vi "RT Functions v03a CMA w TS_Meas.vi"(7 "Function":T5(ring)=enum."CS_Measure", 8 "error in (no error)":errorcluster, 9 "DAQ Trigger":T4={"Trig Source"=0, "Digital Trigger"=FALSE, "Trig Edge"=10171, "Pulse Line"=0, "Pulse On Time"=0} {"Pulse Line" items=["/Line0", "/Line1", "/Line2", "/Line3", "/Line4", "/Line5", "/Line6", "/Line7", "/Line8", "/Line9", "/Line10", "/Line11", "/Line12", "/Line13", "/Line14", "/Line15"]; "Trig Edge" items=["Rising"=10280, "Falling"=10171]; "Trig Source" items=["PFI0", "PFI1", "PFI2", "PFI3", "PFI4", "PFI5", "PFI6", "PFI7", "PFI8", "PFI9", "PFI10", "PFI11", "PFI12", "PFI13", "PFI14", "PFI15"]}, 10 "DAQ Timing":T3={"Number of Samples"=40000, "Samples Per Second"=970000.0, "Sample Mode"=10178, "Timeout (s)"=10.0} {"Sample Mode" items=["Continuous"=10123, "Finite Sample"=10178, "Hardware Timed Single Point"=12522]}, 11 "DAQ Channel":T2={"Channel"=1, "input terminal configuration"=10106, "Input Range Range"=10.0, "Device"="DAQ1"} {"input terminal configuration" items=["default"=-1, "RSE"=10083, "NRSE"=10078, "Differential"=10106, "Pseudodifferential"=12529]; "Input Range Range" items=["+/-10V"=10.0, "+/-5V"=5.0, "+/-2V"=2.0, "+/-1V"=1.0, "+/-0.5V"=0.5, "+/-0.2V"=0.2, "+/-0.1V"=0.1]; "Channel" items=["0"=0, "1"=1, "2"=2, "3"=3, "4"=4, "5"=5, "6"=6, "7"=7, "8"=8, "9"=9, "10"=10, "11"=11, "12"=12, "13"=13, "14"=14, "15"=15, "16"=16, "17"=18, "19"=20, "21"=22, "23"=24, "25"=26, "27"=28, "29"=30, "31"=32]}) -> (0 "error out":errorcluster, 2 "Wfm":waveform(dbl)={"t0"=timestamp(3404415606.9661703 s since 1904-01-01), "dt"=1.0299999999999546e-06, "Y"=array[1600 elements], "attributes"=variant("NI_ChannelName"=variant(string "Voltage"), "NI_UnitDescription"=variant(string "Volts"))}, 3 "Mean":dbl format="%0.2f", 6 "DAQ Pusle":T1)   [LabVIEW 2013]
uses:
  <vilib>/Analysis/baseanly.llb/Mean (DBL).vi
  <vilib>/Waveform/WDTOps.llb/WDT Get Waveform Subset DBL.vi
  <vilib>/Analysis/NI_AALBase.lvlib
panel:
  out "V1_Wfm 2":waveform(dbl)
  out "V2_Wfm 2":waveform(dbl)
  out "V3_Wfm":waveform(dbl)
  out "V2_Wfm":waveform(dbl)
  out "V1_Wfm":waveform(dbl)
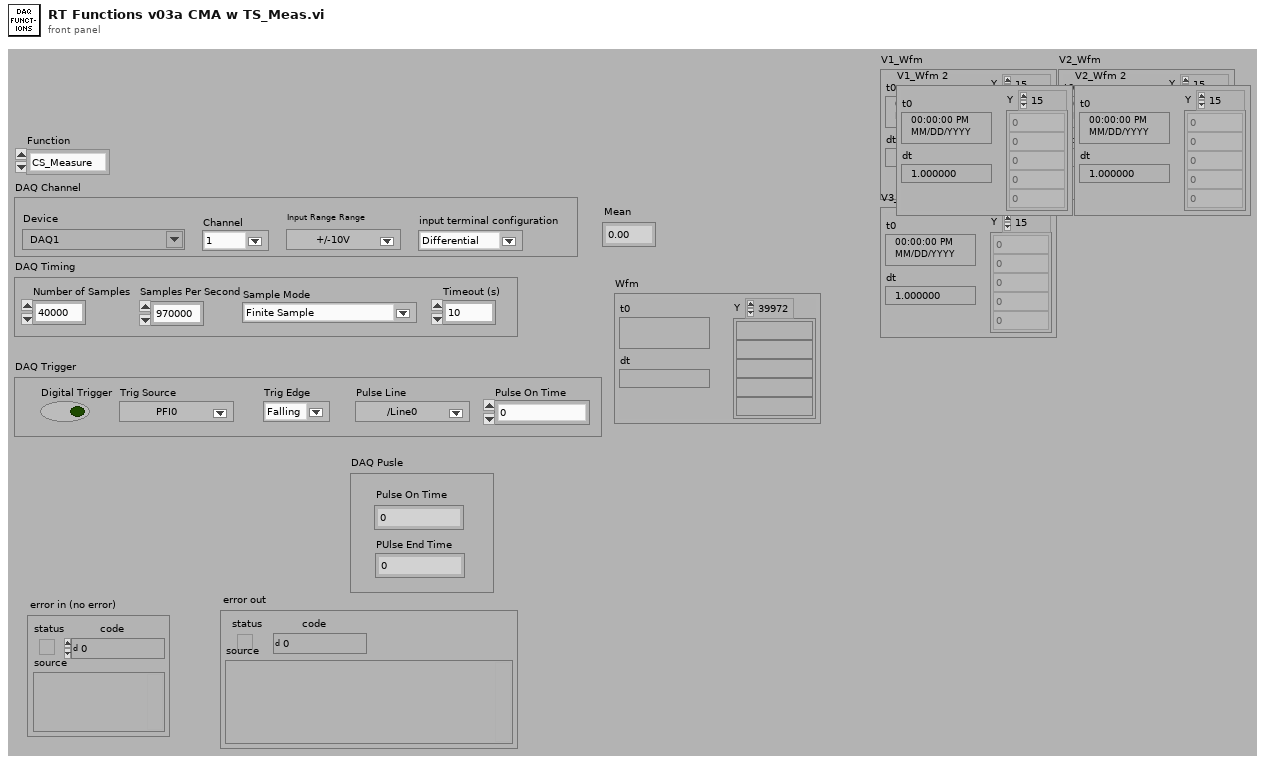
[diagram p1: front panel]
types:
  T1 = cluster{"Pulse On Time":u32, "PUlse End Time":u32}
  T2 = cluster{"Channel":u16, "input terminal configuration":i32, "Input Range Range":dbl, "Device":string}
  T3 = cluster{"Number of Samples":u32, "Samples Per Second":dbl, "Sample Mode":i32, "Timeout (s)":dbl}
  T4 = cluster{"Trig Source":u16, "Digital Trigger":bool, "Trig Edge":i32, "Pulse Line":u16, "Pulse On Time":u32}
  T5 = enum32{"V1 Measure", "V2 Measure", "V3 Measure", "CS_Measure", "TS_Measure", "Pulse On", "Pulse Off"}
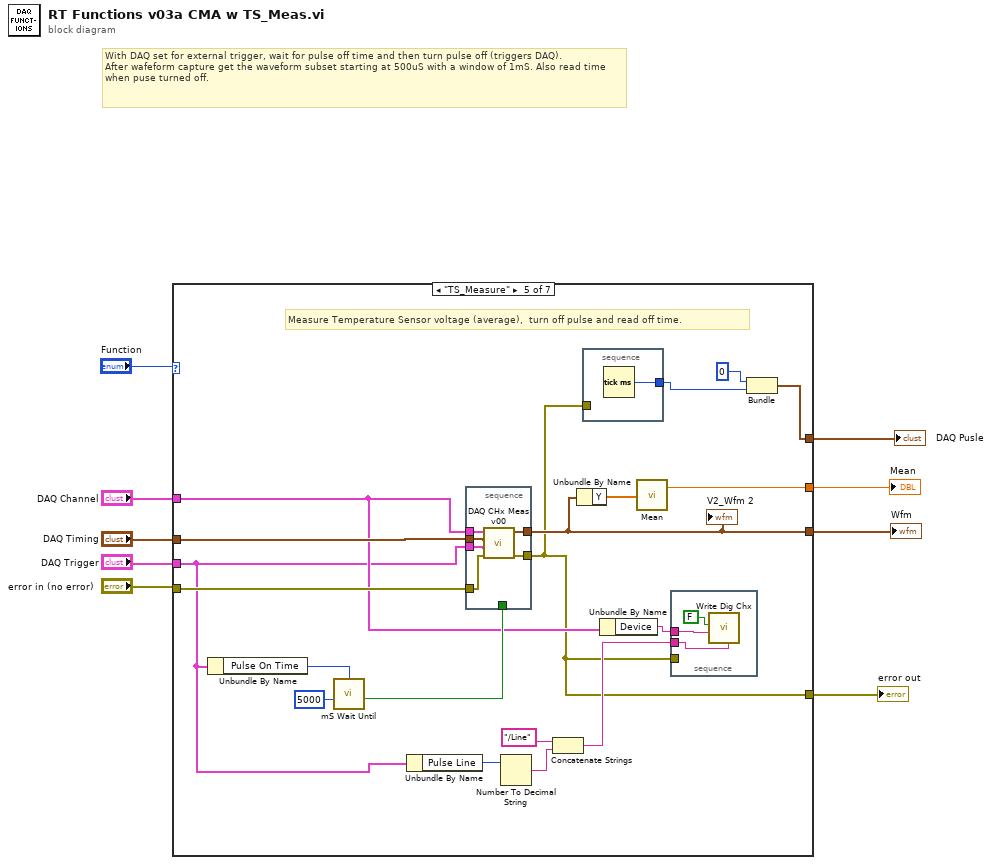
[diagram p0: block diagram]
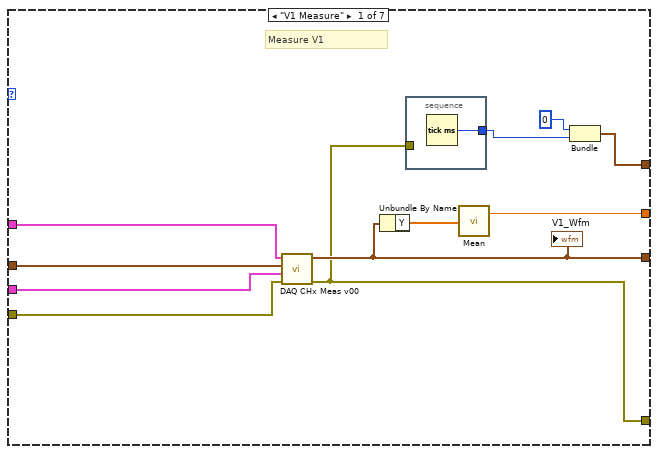
[diagram p2: hidden frame]
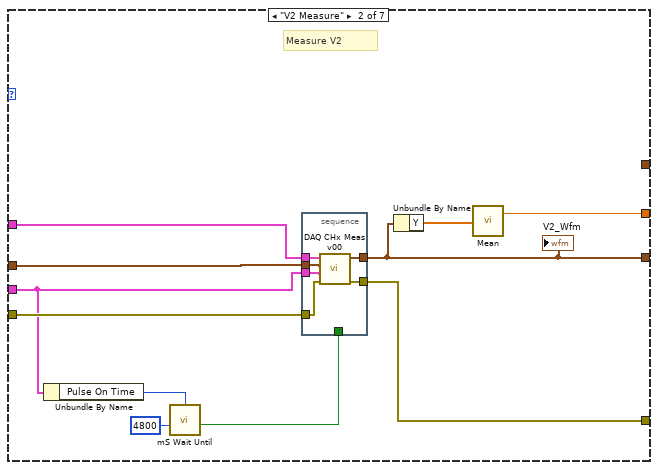
[diagram p3: hidden frame]
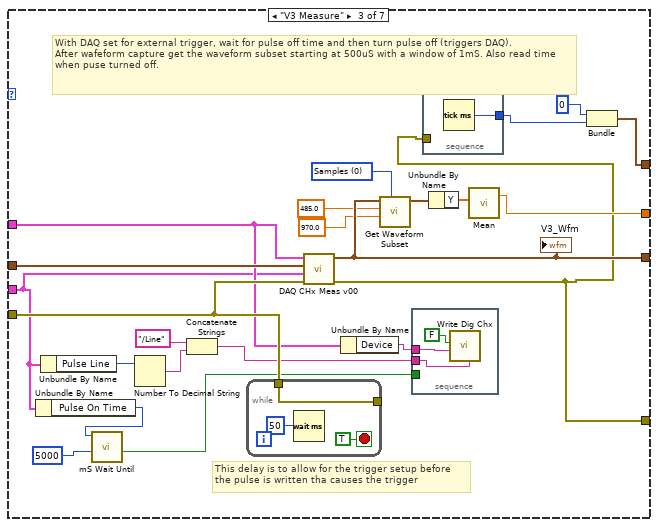
[diagram p4: hidden frame]
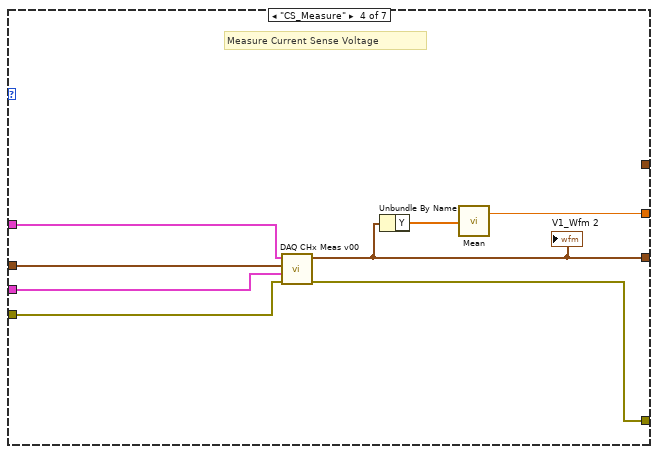
[diagram p5: hidden frame]
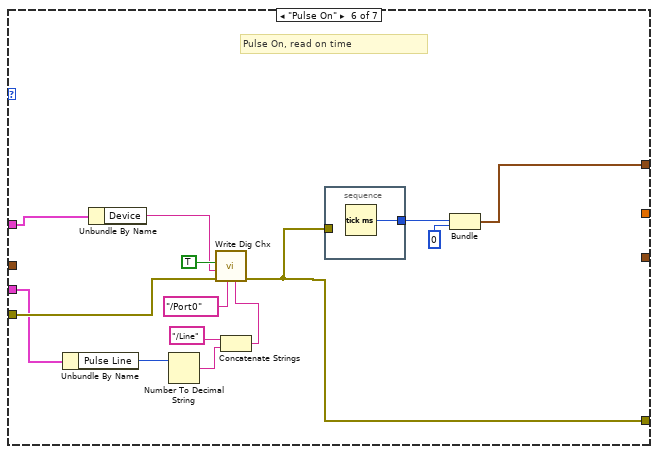
[diagram p6: hidden frame]
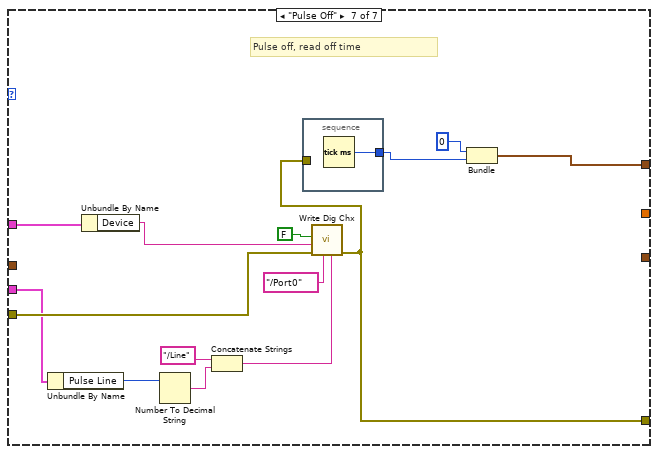
[diagram p7: hidden frame]
diagram:
  # "With DAQ set for external trigger, wait for pulse off time and then turn pulse off (triggers DAQ).\nAfter wafeform capture get the waveform subset starting at 500uS with a window of 1mS. Also read time when puse turned off."
  n1 = case shown="\"TS_Measure\"" "Function" {
    tunnel: "error in (no error)" -> [w20 w31 w58 w76 w95 w118 w133]
    tunnel: [w10 w32 w39 w75 w77 w114 w129] -> w8
    tunnel: "DAQ Channel" -> [w14 w26 w57 w69 w86 w117 w132]
    tunnel: "DAQ Timing" -> [w19 w30 w61 w74 w94 _ _]
    tunnel: "DAQ Trigger" -> [w18 w22 w43 w73 w82 w109 w124]
    tunnel: [w17 w28 w55 w72 w92 _ _] -> w3
    tunnel: [w15 w27 w59 w70 w91 _ _] -> w2
    tunnel: [w11 _ w40 _ w78 w106 w123] -> w1
    frame "V1 Measure" {
      # "Measure V1"
      n2 = call "DAQ CHx Meas v00.vi"("error in"=w20, "DAQ Trigger"=w18, "DAQ Timing"=w19, "DAQ Channel"=w14) -> ("error out"=w10:errorcluster, "Waveform"=w17:waveform(dbl))  [unwired: 6 in]
      "V1_Wfm" <- w17
      n3 = Unbundle By Name(w17) -> ("Y"=w16:dbl[])
      n4 = stacked-sequence {
        tunnel: [w21] -> w13
        tunnel: w10 -> [_]
        frame #0 {
          n5 = Tick Count (ms)() -> (millisecond timer value=w21:u32)
        }
      }
      n6 = call-poly <vilib>:"Mean.vi"("X"=w16) -> ("mean"=w15:dbl)  [unwired: 1 out]
      n7 = Bundle(u32 0, "millisecond timer value"=w13) -> (w11:cluster{u32, "millisecond timer value":u32})  [unwired: 1 in]
    }
    frame "V2 Measure" {
      # "Measure V2"
      n8 = Unbundle By Name(w22) -> ("Pulse On Time"=w23:u32)
      n9 = call "mS Wait Until.vi"("mS Delta"=u16 4800, "mS Start Time"=w23) -> ("Done"=w24:bool)  [unwired: 8 in, 1 out]
      n10 = stacked-sequence {
        tunnel: [w38] -> w32
        tunnel: w31 -> [w37]
        tunnel: w30 -> [w36]
        tunnel: w22 -> [w35]
        tunnel: [w34] -> w28
        tunnel: w26 -> [w33]
        tunnel: w24 -> [_]
        frame #0 {
          n11 = call "DAQ CHx Meas v00.vi"("error in"=w37, "DAQ Trigger"=w35, "DAQ Timing"=w36, "DAQ Channel"=w33) -> ("error out"=w38:errorcluster, "Waveform"=w34:waveform(dbl))  [unwired: 6 in]
        }
      }
      "V2_Wfm" <- w28
      n12 = Unbundle By Name(w28) -> ("Y"=w29:dbl[])
      n13 = call-poly <vilib>:"Mean.vi"("X"=w29) -> ("mean"=w27:dbl)  [unwired: 1 out]
    }
    frame "V3 Measure" {
      w54 = u16 0 items=["Samples", "Relative Time"] ("start/duration format")
      # "With DAQ set for external trigger, wait for pulse off time and then turn pulse off (triggers DAQ).\nAfter wafeform capture get the waveform subset starting at 500uS with a window of 1mS. Also read time when puse turned off."
      # "This delay is to allow for the trigger setup before\nthe pulse is written tha causes the trigger"
      n14 = Unbundle By Name(w43) -> ("Pulse On Time"=w48:u32)
      n15 = Unbundle By Name(w43) -> ("Pulse Line"=w47:u16)
      n16 = call "mS Wait Until.vi"("mS Delta"=u16 5000, "mS Start Time"=w48) -> ("Done"=w49:bool)  [unwired: 8 in, 1 out]
      n17 = Number To Decimal String(number=w47) -> (decimal integer string=w46:string)  [unwired: 1 in]
      n18 = Concatenate Strings("/Line", w46) -> (w44:string)
      n19 = while {
        tunnel: w58 -> [w66]
        tunnel: [w66] -> _
        stop <- TRUE stop-if-true
        n20 = Wait (ms)(milliseconds to wait=u32 50) -> ()  [unwired: 1 out]
      }
      n21 = call "DAQ CHx Meas v00.vi"("error in"=w58, "DAQ Trigger"=w43, "DAQ Timing"=w61, "DAQ Channel"=w57) -> ("error out"=w39:errorcluster, "Waveform"=w55:waveform(dbl))  [unwired: 6 in]
      "V3_Wfm" <- w55
      n22 = Unbundle By Name(w57) -> ("Device"=w56:string)
      n23 = call-poly <vilib>:"Get Waveform Subset.vi"("start/duration format"=w54, "duration"=970.0, "start samples/time"=485.0, "waveform in"=w55) -> ("waveform out"=w51:waveform(dbl))  [unwired: 2 in, 3 out]
      n24 = stacked-sequence {
        tunnel: w56 -> [w64]
        tunnel: w44 -> [w63]
        tunnel: w49 -> [_]
        frame #0 {
          n25 = call "Write Dig Chx.vi"("Line"=w63, "Device"=w64, "Ch Value"=FALSE) -> ()  [unwired: 8 in, 1 out]
        }
      }
      n26 = stacked-sequence {
        tunnel: [w62] -> w41
        tunnel: w39 -> [_]
        frame #0 {
          n27 = Tick Count (ms)() -> (millisecond timer value=w62:u32)
        }
      }
      n28 = Unbundle By Name(w51) -> ("Y"=w60:dbl[])
      n29 = call-poly <vilib>:"Mean.vi"("X"=w60) -> ("mean"=w59:dbl)  [unwired: 1 out]
      n30 = Bundle(u32 0, "millisecond timer value"=w41) -> (w40:cluster{u32, "millisecond timer value":u32})  [unwired: 1 in]
    }
    frame "CS_Measure" {
      # "Measure Current Sense Voltage"
      n31 = call "DAQ CHx Meas v00.vi"("error in"=w76, "DAQ Trigger"=w73, "DAQ Timing"=w74, "DAQ Channel"=w69) -> ("error out"=w75:errorcluster, "Waveform"=w72:waveform(dbl))  [unwired: 6 in]
      "V1_Wfm 2" <- w72
      n32 = Unbundle By Name(w72) -> ("Y"=w71:dbl[])
      n33 = call-poly <vilib>:"Mean.vi"("X"=w71) -> ("mean"=w70:dbl)  [unwired: 1 out]
    }
    frame "TS_Measure" {
      # "Measure Temperature Sensor voltage (average),  turn off pulse and read off time."
      n34 = Unbundle By Name(w82) -> ("Pulse On Time"=w88:u32)
      n35 = call "mS Wait Until.vi"("mS Delta"=u16 5000, "mS Start Time"=w88) -> ("Done"=w89:bool)  [unwired: 8 in, 1 out]
      n36 = Unbundle By Name(w82) -> ("Pulse Line"=w83:u16)
      n37 = stacked-sequence {
        tunnel: [w105] -> w77
        tunnel: w95 -> [w104]
        tunnel: w94 -> [w103]
        tunnel: w82 -> [w102]
        tunnel: [w101] -> w92
        tunnel: w86 -> [w100]
        tunnel: w89 -> [_]
        frame #0 {
          n38 = call "DAQ CHx Meas v00.vi"("error in"=w104, "DAQ Trigger"=w102, "DAQ Timing"=w103, "DAQ Channel"=w100) -> ("error out"=w105:errorcluster, "Waveform"=w101:waveform(dbl))  [unwired: 6 in]
        }
      }
      "V2_Wfm 2" <- w92
      n39 = Number To Decimal String(number=w83) -> (decimal integer string=w84:string)  [unwired: 1 in]
      n40 = Concatenate Strings("/Line", w84) -> (w81:string)
      n41 = Unbundle By Name(w92) -> ("Y"=w93:dbl[])
      n42 = stacked-sequence {
        tunnel: [w96] -> w80
        tunnel: w77 -> [_]
        frame #0 {
          n43 = Tick Count (ms)() -> (millisecond timer value=w96:u32)
        }
      }
      n44 = Unbundle By Name(w86) -> ("Device"=w87:string)
      n45 = call-poly <vilib>:"Mean.vi"("X"=w93) -> ("mean"=w91:dbl)  [unwired: 1 out]
      n46 = stacked-sequence {
        tunnel: w87 -> [w98]
        tunnel: w81 -> [w97]
        tunnel: w77 -> [_]
        frame #0 {
          n47 = call "Write Dig Chx.vi"("Line"=w97, "Device"=w98, "Ch Value"=FALSE) -> ()  [unwired: 8 in, 1 out]
        }
      }
      n48 = Bundle(u32 0, "millisecond timer value"=w80) -> (w78:cluster{u32, "millisecond timer value":u32})  [unwired: 1 in]
    }
    frame "Pulse On" {
      # "Pulse On, read on time"
      n49 = Unbundle By Name(w109) -> ("Pulse Line"=w111:u16)
      n50 = Unbundle By Name(w117) -> ("Device"=w116:string)
      n51 = Number To Decimal String(number=w111) -> (decimal integer string=w112:string)  [unwired: 1 in]
      n52 = Concatenate Strings("/Line", w112) -> (w110:string)
      n53 = call "Write Dig Chx.vi"("Line"=w110, "Port"="/Port0", "error in"=w118, "Device"=w116, "Ch Value"=TRUE) -> ("error out"=w114:errorcluster)  [unwired: 6 in]
      n54 = stacked-sequence {
        tunnel: w114 -> [_]
        tunnel: [w120] -> w108
        frame #0 {
          n55 = Tick Count (ms)() -> (millisecond timer value=w120:u32)
        }
      }
      n56 = Bundle("millisecond timer value"=w108, u32 0) -> (w106:cluster{"millisecond timer value":u32, u32})  [unwired: 1 in]
    }
    frame "Pulse Off" {
      # "Pulse off, read off time"
      n57 = Unbundle By Name(w124) -> ("Pulse Line"=w126:u16)
      n58 = Unbundle By Name(w132) -> ("Device"=w131:string)
      n59 = Number To Decimal String(number=w126) -> (decimal integer string=w127:string)  [unwired: 1 in]
      n60 = Concatenate Strings("/Line", w127) -> (w125:string)
      n61 = call "Write Dig Chx.vi"("Line"=w125, "Port"="/Port0", "error in"=w133, "Device"=w131, "Ch Value"=FALSE) -> ("error out"=w129:errorcluster)  [unwired: 6 in]
      n62 = stacked-sequence {
        tunnel: w129 -> [_]
        tunnel: [w135] -> w122
        frame #0 {
          n63 = Tick Count (ms)() -> (millisecond timer value=w135:u32)
        }
      }
      n64 = Bundle(u32 0, "millisecond timer value"=w122) -> (w123:cluster{u32, "millisecond timer value":u32})  [unwired: 1 in]
    }
  }
  "error out" <- w8
  "Wfm" <- w3
  "Mean" <- w2
  "DAQ Pusle" <- w1
